vi "SPARK Set Parameter.vi"   [LabVIEW 2023]
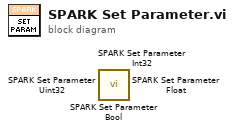
[diagram p0: block diagram]
diagram:
  n1 = call <vilib>:"SPARK Set Parameter Bool.vi"() -> ()  [unwired: 10 in, 2 out]
  n2 = call <vilib>:"SPARK Set Parameter Int32.vi"() -> ()  [unwired: 10 in, 2 out]
  n3 = call <vilib>:"SPARK Set Parameter Uint32.vi"() -> ()  [unwired: 10 in, 2 out]
  n4 = call <vilib>:"SPARK Set Parameter Float.vi"() -> ()  [unwired: 10 in, 2 out]
